vi "DAC Init Results.vi"(8 "error in":errorcluster, 9 "Log Details?":bool, 10 "tdms file":refnum<k34>, 11 "DAC ADV in":refnum<class "DAC ADV.lvclass">) -> (0 "error out":errorcluster, 2 "tdms file out":refnum<k34>)   [LabVIEW 2019, in "DAC.lvlib" / "DAC ADV.lvclass"]
uses:
  DAC ADV.lvclass
  DAC.lvclass
  C:/Users/wg/Documents/LV_Projects/test-stand/App/DAC/DAC.lvclass
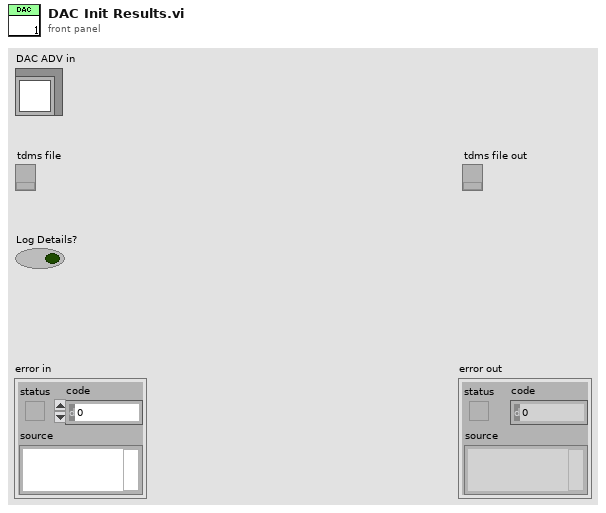
[diagram p1: front panel]
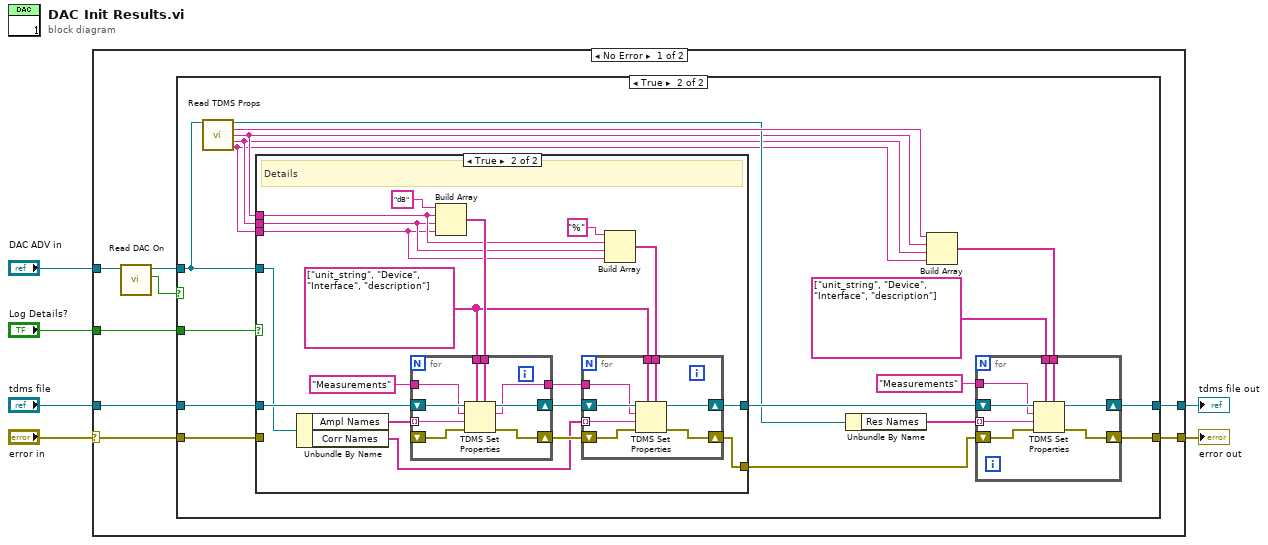
[diagram p0: block diagram]
diagram:
  n1 = case shown="No Error" "error in" {
    selector: "error in" -> [w8 w80]
    tunnel: [w12 w80] -> w3
    tunnel: "DAC ADV in" -> [w11 _]
    tunnel: "tdms file" -> [w14 w79]
    tunnel: [w13 w79] -> w2
    tunnel: "Log Details?" -> [w7 _]
    frame No Error {
      n2 = call "Read DAC On.vi"("DAC in"=w11) -> ("DAC On"=w9:bool, "DAC out"=w10:refnum<class "DAC ADV.lvclass">)  [unwired: 8 in, 1 out]
      n3 = case shown="True" w9 {
        tunnel: w14 -> [w16 w29]
        tunnel: [w16 w33] -> w13
        tunnel: [w15 w32] -> w12
        tunnel: w10 -> [_ w24]
        tunnel: w8 -> [w15 w25]
        tunnel: w7 -> [_ w30]
        frame False {
        }
        frame True {
          n4 = call "Read TDMS Props.vi"("DAC in"=w24) -> ("DAC out"=w21:refnum<class "DAC ADV.lvclass">, "Result Unit"=w22:string, "DAC Device"=w19:string, "DAC IO"=w18:string, "DAC Description"=w17:string)  [unwired: 10 in]
          n5 = case shown="True" w30 {
            tunnel: w29 -> [w35 w52]
            tunnel: [w35 w46] -> w28
            tunnel: w24 -> [_ w51]
            tunnel: [w34 w48] -> w26
            tunnel: w25 -> [w34 _]
            tunnel: w19 -> [_ w38]
            tunnel: w18 -> [_ w37]
            tunnel: w17 -> [_ w36]
            frame False {
            }
            frame True {
              w39 = string[] ["unit_string", "Device", "Interface", "description"] ("property names")
              # "Details"
              n6 = Unbundle By Name(w51) -> ("Ampl Names"=w41:string[], "Corr Names"=w40:string[])
              n7 = Build Array("dB" ("element"), w38, w37, w36) -> (w53:string[])
              n8 = for {
                tunnel: w39 -> [w69]
                tunnel: w53 -> [w68]
                shift-right: [w67] -> w47
                shift-left: w52 -> [w70]
                tunnel: "Measurements" ("group name in (Untitled)") -> [w65]
                shift-right: [w66] -> w49
                shift-left: _ -> [w64]
                tunnel: w41 -> [w63] mode=indexing
                tunnel: [w62] -> w44
                n9 = TDMS Set Properties(5:w68, 7:w69, 8:w64, 9:w63, 10:w65, 11:w70) -> (0:w66:errorcluster, 2:w62:string, 3:w67:refnum<k34>)  [unwired: 1 out]
              }
              n10 = Build Array("%" ("element"), w38, w37, w36) -> (w45:string[])
              n11 = for {
                tunnel: w39 -> [w60]
                tunnel: w45 -> [w59]
                shift-right: [w58] -> w46
                shift-left: w47 -> [w61]
                tunnel: w44 -> [w56]
                shift-right: [w57] -> w48
                shift-left: w49 -> [w55]
                tunnel: w40 -> [w54] mode=indexing
                n12 = TDMS Set Properties(5:w59, 7:w60, 8:w55, 9:w54, 10:w56, 11:w61) -> (0:w57:errorcluster, 3:w58:refnum<k34>)  [unwired: 2 out]
              }
            }
          }
          n13 = Unbundle By Name(w21) -> ("Res Names"=w31:string[])
          n14 = Build Array(w22, w19, w18, w17) -> (w20:string[])
          n15 = for {
            tunnel: w31 -> [w77] mode=indexing
            tunnel: string[] ["unit_string", "Device", "Interface", "description"] ("property names") -> [w76]
            tunnel: w20 -> [w75]
            shift-right: [w74] -> w33
            shift-left: w28 -> [w78]
            tunnel: "Measurements" ("group name in (Untitled)") -> [w72]
            shift-right: [w73] -> w32
            shift-left: w26 -> [w71]
            n16 = TDMS Set Properties(5:w75, 7:w76, 8:w71, 9:w77, 10:w72, 11:w78) -> (0:w73:errorcluster, 3:w74:refnum<k34>)  [unwired: 2 out]
          }
        }
      }
    }
    frame Error {
    }
  }
  "error out" <- w3
  "tdms file out" <- w2
